vi "Encode Relay ID.vi"(8 "error in (no error)":errorcluster, 11 "Relay ID":T1 {"Serial Number" format="%06x"}) -> (0 "error out":errorcluster, 3 "Encoded ID":u8[](array[numeric]) format="%.0x")   [LabVIEW 2021, in "USB Relay Control.lvlib"]
uses:
  USB Relay Control.lvlib
  typedef/Relay ID.ctl
  <vilib>/CIF Foundation/CIF Utilities/DataTypes/Typedef/Endian.ctl
  typedef/Errors.ctl
  Add USB Relay Error Core.vi
  <vilib>/CIF Foundation/CIF Utilities/DataTypes/DataTypes_CIF_U.lvlib
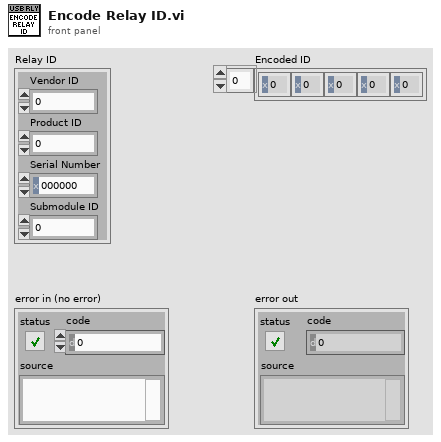
[diagram p1: front panel]
types:
  T1 = typedef "USB Relay Control.lvlib/Relay ID.ctl" = cluster{"Vendor ID":u8, "Product ID":u8, "Serial Number":u32, "Submodule ID":u8}
  T2 = typedef "USB Relay Control.lvlib/Errors.ctl" = enum16{"Invalid ID"}
  T3 = typedef "DataTypes_CIF_U.lvlib/Endian.ctl" = enum16{"Little Endian", "Big Endian"}
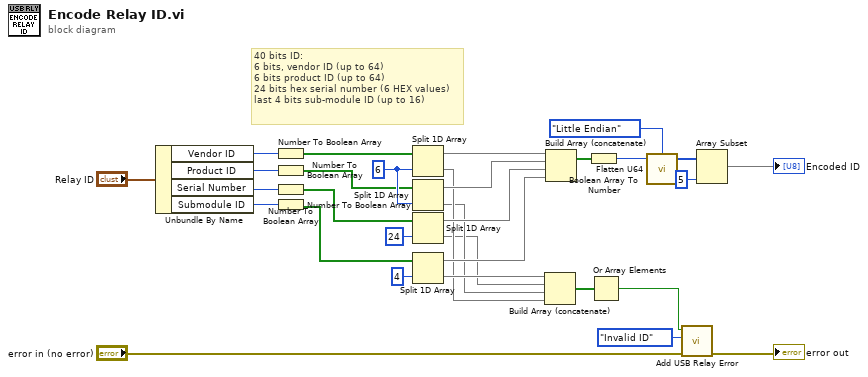
[diagram p0: block diagram]
diagram:
  w23 = 6 ("index")
  # "40 bits ID:\n6 bits, vendor ID (up to 64)\n6 bits product ID (up to 64)\n24 bits hex serial number (6 HEX values)\nlast 4 bits sub-module ID (up to 16)"
  n1 = Unbundle By Name("Relay ID") -> ("Vendor ID"=w28:u8, "Product ID"=w29:u8, "Serial Number"=w30:u32, "Submodule ID"=w31:u8)
  n2 = Number To Boolean Array(number=w28) -> (Boolean array=w24:bool[])
  n3 = Number To Boolean Array(number=w29) -> (Boolean array=w22:bool[])
  n4 = Number To Boolean Array(number=w30) -> (Boolean array=w17:bool[])
  n5 = Number To Boolean Array(number=w31) -> (Boolean array=w21:bool[])
  n6 = Split 1D Array(array=w24, index=w23) -> (first subarray=w27:bool[], second subarray=w8:bool[])
  n7 = Split 1D Array(array=w22, index=w23) -> (first subarray=w25:bool[], second subarray=w7:bool[])
  n8 = Split 1D Array(array=w17, index=24) -> (first subarray=w16:bool[], second subarray=w6:bool[])
  n9 = Split 1D Array(array=w21, index=4) -> (first subarray=w19:bool[], second subarray=w9:bool[])
  n10 = Build Array (concatenate)(w9, w6, w7, w8) -> (w5:bool[])
  n11 = Build Array (concatenate)(w27, w25, w16, w19) -> (w26:bool[])
  n12 = Boolean Array To Number(Boolean array=w26) -> (number=w18:u64)
  n13 = Or Array Elements(Boolean array=w5) -> (logical OR=w4:bool)
  n14 = call <vilib>:"Flatten U64.vi"("U64"=w18, "Endian"=Endian."Little Endian") -> ("Flat Data"=w13:u8[])  [unwired: 3 in]
  n15 = call "Add USB Relay Error.vi"("error in (no error)"="error in (no error)", "Error"=Errors."Invalid ID", "Insert Error"=w4) -> ("error out"=→"error out":errorcluster)  [unwired: 8 in]
  n16 = Array Subset(array=w13, length=5) -> (→"Encoded ID":u8[])  [unwired: 1 in]
